vi "Apply Setpoints.vi"(8 "error in":errorcluster, 10 "setpoints":T1[](array[typedef]), 11 "Rig in":refnum<class "Rig.lvclass">) -> (0 "error out":errorcluster, 3 "Rig out":refnum<class "Rig.lvclass">)   [LabVIEW 2026, in "Rig.lvclass"]
doc: "Applies setpoints to the rig. Dynamic dispatch, must be overridden by every rig plug-in. The base implementation does nothing and passes the object and the error through."
uses:
  Rig.lvclass
  Rig.lvclass/Rig.ctl
  Typedefs/Channel Value.ctl
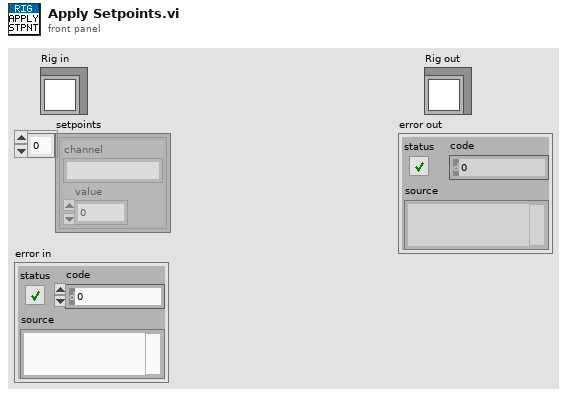
[diagram p1: front panel]
types:
  T1 = typedef "Channel Value.ctl" = cluster{"channel":string, "value":dbl}
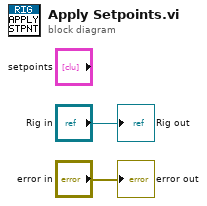
[diagram p0: block diagram]
diagram:
  "Rig out" <- "Rig in"
  "error out" <- "error in"
